vi "Obtain Request Events.vi"(8 "error in":errorcluster, 10 "Create New? (F)":bool, 11 "Module ID":i32=-1) -> (0 "error out":errorcluster, 2 "Core Request Events":T1)   [LabVIEW 2026, in "Core.lvlib"]
doc: "This VI Obtains/Creates the Requests events that will be used for other modules to communicate with the module that owns this VI. These Requests events will be accessed only via Public API methods for this module.\n\n<b>NOTE</b>: The contents of this VI are automatically generated and modified by the <b>Tools > DQMH Consortium > DQMH</b> utilities. Consider using those utilities instead of making your own modifications to this VI.\n_____\nBased on DQMH Dev Tools: Project Template 7.1.2.1547."
uses:
  Core.lvlib
  Request Events--cluster.ctl
  Stop Argument--cluster.ctl
  Show Panel Argument--cluster.ctl
  Hide Panel Argument--cluster.ctl
  Show Diagram Argument--cluster.ctl
  Get Module Execution Status Argument--cluster.ctl
  Resubscribe to Cloneable Argument--cluster.ctl
  replay/Replay/src/Libraries/Replay/Broadcast Events--cluster.ctl
  replay/Replay/src/Libraries/Replay/Did Init Argument--cluster.ctl
  replay/Replay/src/Libraries/Replay/Status Updated Argument--cluster.ctl
  replay/Replay/src/Libraries/Replay/Error Reported Argument--cluster.ctl
  replay/Replay/src/Libraries/Replay/Stop Argument--cluster.ctl
  replay/Replay/src/Libraries/Replay/Get Module Execution Status Argument--cluster.ctl
  replay/Replay/src/Libraries/Replay/Replay Finished Processing User Events Argument--cluster.ctl
  replay/Replay/src/Libraries/Replay/Load UserEvents (Reply Payload)--cluster.ctl
  replay/Replay/src/Libraries/User Events Metadata.ctl
  LaunchReplayModule Argument--cluster.ctl
  Local Instance Request Events--cluster.ctl
  Set Record Run ID Argument--cluster.ctl
  Record Run ID Argument--cluster.ctl
  Record Run ID (Reply Payload)--cluster.ctl
  replay/Replay/src/Libraries/Replay/Replay.lvlib
  Local Instance Events SEQ/Local Instance Events SEQ.lvlib
panel:
  # "NOTE: The contents of this VI are automatically generated and modified by the Tools > DQMH Consortium > DQMH utilities. Consider using those utilities instead of making your own modifications to this VI."
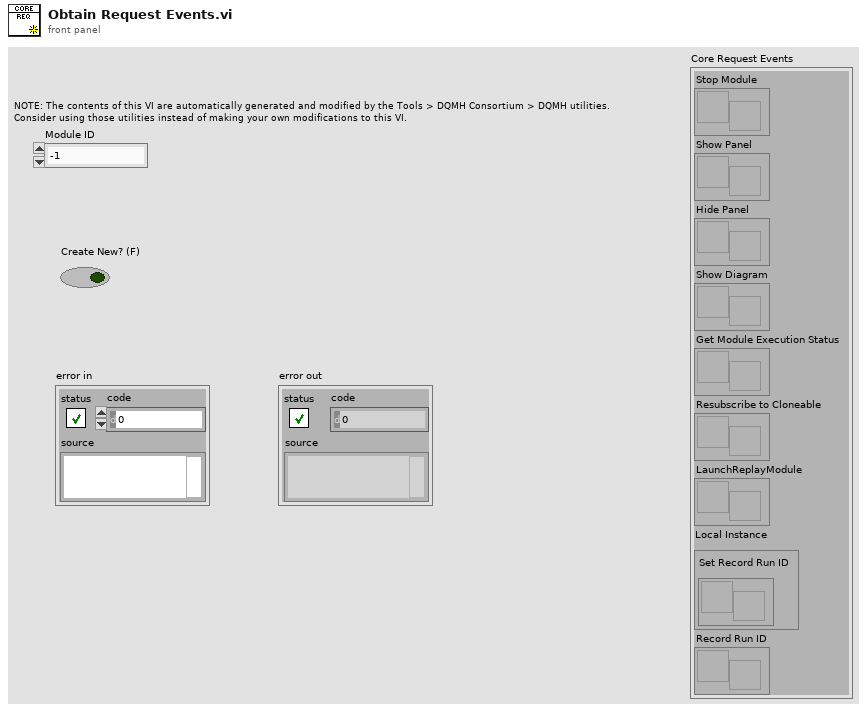
[diagram p1: front panel]
types:
  T1 = typedef "Core.lvlib/Request Events--cluster.ctl" = cluster{"Stop Module":refnum<user-event>, "Show Panel":refnum<user-event>, "Hide Panel":refnum<user-event>, "Show Diagram":refnum<user-event>, "Get Module Execution Status":refnum<user-event>, "Resubscribe to Cloneable":refnum<user-event>, "LaunchReplayModule":refnum<user-event>, "Local Instance":T2, "Record Run ID":refnum<user-event>}
  T2 = typedef "Core.lvlib/Local Instance Request Events--cluster.ctl" = cluster{"Set Record Run ID":refnum<user-event>}
  T3 = typedef "Core.lvlib/Record Run ID Argument--cluster.ctl" = cluster{"Module ID":i32, "Record Run ID":string, "Wait Notifier":refnum<notifier>, "wait for reply":bool}
  T4 = typedef "Core.lvlib/LaunchReplayModule Argument--cluster.ctl" = cluster{"Module ID":i32, "Run ID":string}
  T5 = typedef "Core.lvlib/Resubscribe to Cloneable Argument--cluster.ctl" = cluster{"Module ID":i32, "Replay Broadcast Events":T6}
  T6 = typedef "Replay.lvlib/Broadcast Events--cluster.ctl" = cluster{"Module Did Init":refnum<user-event>, "Status Updated":refnum<user-event>, "Error Reported":refnum<user-event>, "Module Did Stop":refnum<user-event>, "Update Module Execution Status":refnum<user-event>, "Replay Finished Processing User Events":refnum<user-event>, "User Events Metadata":refnum<user-event>}
  T7 = typedef "Core.lvlib/Get Module Execution Status Argument--cluster.ctl" = cluster{"Module ID":i32, "Running?":bool}
  T8 = typedef "Core.lvlib/Show Diagram Argument--cluster.ctl" = cluster{"Module ID":i32, "Debug?":bool}
  T9 = typedef "Core.lvlib/Show Panel Argument--cluster.ctl" = cluster{"Module ID":i32, "Show Panel?":bool}
  T10 = typedef "Core.lvlib/Hide Panel Argument--cluster.ctl" = cluster{"Module ID":i32, "Hide Panel?":bool}
  T11 = typedef "Core.lvlib/Stop Argument--cluster.ctl" = cluster{"Module ID":i32, "Origin":string, "Exit via Stop Module Req?":bool, "Wait for Module to stop?":bool}
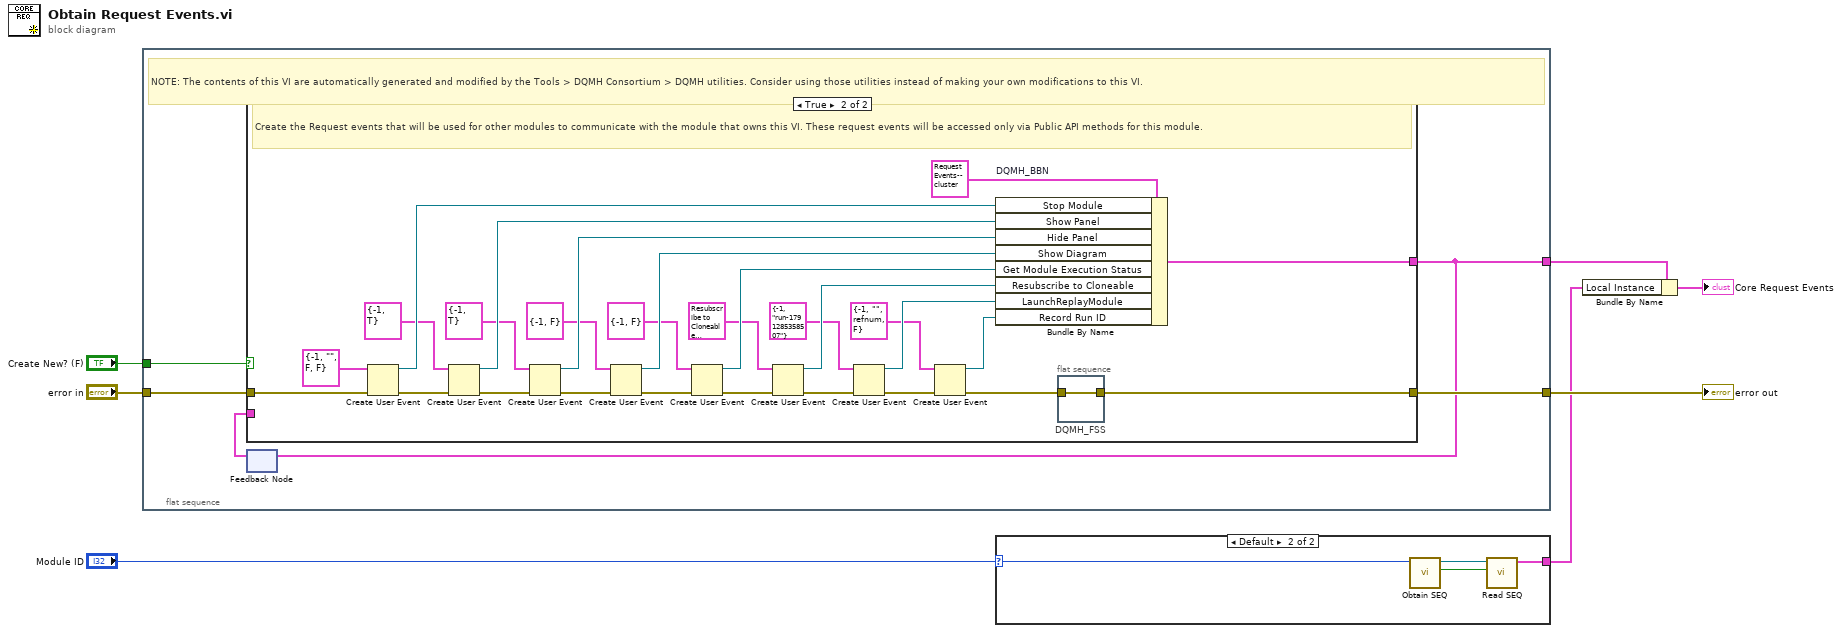
[diagram p0: block diagram]
diagram:
  n1 = flat-sequence {
    tunnel: [w12] -> w7
    tunnel: "error in" -> [w11]
    tunnel: [w9] -> w3
    tunnel: "Create New? (F)" -> [w8]
    frame #0 {
      # "NOTE: The contents of this VI are automatically generated and modified by the Tools > DQMH Consortium > DQMH utilities. Consider using those utilities instead of making your own modifications to this VI."
      n2 = feedback #1() -> (w10:T1)  [unwired: 1 in]
      n3 = case shown="True" w8 {
        tunnel: [w13 w30] -> w12
        tunnel: w11 -> [w13 w42]
        tunnel: [w14 w39] -> w9
        tunnel: w10 -> [w14 _]
        frame False {
        }
        frame True {
          # "Create the Request events that will be used for other modules to communicate with the module that owns this VI. These request events will be accessed only via Public API methods for this module."
          n4 = Create User Event(user event datatype=T11 {"Module ID"=-1, "Origin"="", "Exit via Stop Module Req?"=FALSE, "Wait for Module to stop?"=FALSE} ("Stop Argument"), error in=w42) -> (user event=w40:refnum<user-event>, error out=w37:errorcluster)
          n5 = Create User Event(user event datatype=T9 {"Module ID"=-1, "Show Panel?"=TRUE} ("Show Panel Argument"), error in=w37) -> (user event=w36:refnum<user-event>, error out=w34:errorcluster)
          n6 = Create User Event(user event datatype=T10 {"Module ID"=-1, "Hide Panel?"=TRUE} ("Hide Panel"), error in=w34) -> (user event=w33:refnum<user-event>, error out=w32:errorcluster)
          n7 = Create User Event(user event datatype=T8 {"Module ID"=-1, "Debug?"=FALSE} ("Show Diagram Argument"), error in=w32) -> (user event=w28:refnum<user-event>, error out=w29:errorcluster)
          n8 = Create User Event(user event datatype=T7 {"Module ID"=-1, "Running?"=FALSE} ("Get Module Execution Status Argument"), error in=w29) -> (user event=w25:refnum<user-event>, error out=w26:errorcluster)
          n9 = Create User Event(user event datatype=T5 {"Module ID"=-1, "Replay Broadcast Events"={"Module Did Init"=refnum, "Status Updated"=refnum, "Error Reported"=refnum, "Module Did Stop"=refnum, "Update Module Execution Status"=refnum, "Replay Finished Processing User Events"=refnum, "User Events Metadata"=refnum}} ("Resubscribe to Cloneable Argument"), error in=w26) -> (user event=w22:refnum<user-event>, error out=w23:errorcluster)
          n10 = Create User Event(user event datatype=T4 {"Module ID"=-1, "Run ID"="run-1791285358507"} ("LaunchReplayModule Argument"), error in=w23) -> (user event=w19:refnum<user-event>, error out=w20:errorcluster)
          n11 = Create User Event(user event datatype=T3 {"Module ID"=-1, "Record Run ID"="", "Wait Notifier"=refnum, "wait for reply"=FALSE} ("Record Run ID Argument"), error in=w20) -> (user event=w16:refnum<user-event>, error out=w17:errorcluster)
          n12 = Bundle By Name "DQMH_BBN"(cluster=T1 {"Stop Module"=refnum, "Show Panel"=refnum, "Hide Panel"=refnum, "Show Diagram"=refnum, "Get Module Execution Status"=refnum, "Resubscribe to Cloneable"=refnum, "LaunchReplayModule"=refnum, "Local Instance"={"Set Record Run ID"=refnum}, "Record Run ID"=refnum} ("output cluster"), "Stop Module"=w40, "Show Panel"=w36, "Hide Panel"=w33, "Show Diagram"=w28, "Get Module Execution Status"=w25, "Resubscribe to Cloneable"=w22, "LaunchReplayModule"=w19, "Record Run ID"=w16) -> (w39:T1)
          n13 = flat-sequence "DQMH_FSS" {
            tunnel: w17 -> [w43]
            tunnel: [w43] -> w30
            frame #0 {
            }
          }
        }
      }
      n14 = feedback-in #1(w9) -> ()
    }
  }
  n15 = case shown="Default" "Module ID" {
    selector: "Module ID" -> [_ w45]
    tunnel: [_ w44] -> w2
    frame -1 {
    }
    frame Default {
      n16 = call "Obtain SEQ.vi"("Module ID"=w45) -> ("Created New?"=w46:bool, "Local Instance Event SEQ"=w47:refnum<queue>)  [unwired: 8 in, 1 out]
      n17 = call "Read SEQ.vi"("Created New?"=w46, "Local Instance Event SEQ"=w47) -> ("Local Instance Request Events"=w44:T2)  [unwired: 8 in, 1 out]
    }
  }
  n18 = Bundle By Name(cluster=w3, "Local Instance"=w2) -> (→"Core Request Events":T1)
  "error out" <- w7
